vi "Test Filter.vi"() -> ()   [LabVIEW 2021]
uses:
  typedef/CAN Filter.ctl
  <vilib>/CIF Foundation/CIF PCAP Parse and Build/Typedef/Format Specific/Socket CAN Header.ctl
  CAN_RW_CORE.lvclass/CAN_RW_CORE.ctl
  CAN_RW_CORE.lvclass
  <vilib>/CIF Foundation/CIF PCAP Parse and Build/pcap_Parse_Build_CIF.lvclass
panel:
  in  "CAN Header in":T1 {"CANID and Flags" format="%.0x"; "FD Flags" format="%.0x"}
  out "Valid":bool
  in  "Filter":T2={"Allow List (ID)"=[], "Deny List (ID)"=[120, 2]} {"Deny List (ID)" format="%.0x"; "Allow List (ID)" format="%.0x"}
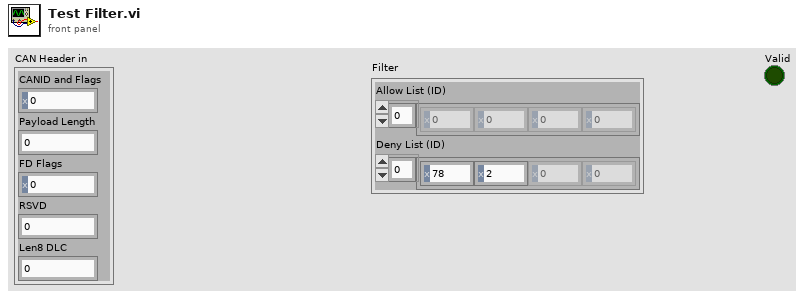
[diagram p1: front panel]
types:
  T1 = typedef "pcap_Parse_Build_CIF.lvclass/Socket CAN Header.ctl" = cluster{"CANID and Flags":u32, "Payload Length":u8, "FD Flags":u8, "RSVD":u8, "Len8 DLC":u8}
  T2 = typedef "CAN_RW_CORE.lvclass/CAN Filter.ctl" = cluster{"Allow List (ID)":u32[], "Deny List (ID)":u32[]}
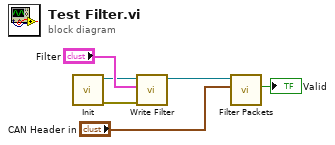
[diagram p0: block diagram]
diagram:
  n1 = call "Init.vi"() -> ("error out"=w3:errorcluster, "CAN_RW_CORE out"=w4:refnum<class "CAN_RW_CORE.lvclass">)  [unwired: 10 in]
  n2 = call "Write Filter.vi"("error in (no error)"=w3, "Filter"="Filter", "CAN_RW_CORE in"=w4) -> ("CAN_RW_CORE out"=w5:refnum<class "CAN_RW_CORE.lvclass">)  [unwired: 7 in, 1 out]
  n3 = call "Filter Packets.vi"("CAN Header in"="CAN Header in", "CAN_RW_CORE"=w5) -> ("Valid"=→"Valid":bool)  [unwired: 9 in]
